vi "Get Username and Password.vi"(8 "error in":errorcluster, 11 "Item Ref in":T1 format="%.0x") -> (0 "error out":errorcluster, 1 "password":string, 2 "username":string, 3 "Item Ref out":T1 format="%.0x")   [LabVIEW 2024, in "SEECD System Explorer.lvlib"]
uses:
  NationalInstruments.VeriStand.SystemDefinitionAPI
  SEECD System Explorer.lvlib
  <vilib>/NI VeriStand/Custom Device Tools/Custom Device Utility Library/Custom Device Utility Library.lvlib
  <vilib>/NI VeriStand/Custom Device Offline API/Custom Device Offline API.lvlib
  <vilib>/NI VeriStand/Custom Device API/Custom Device Item Ref.ctl
  <vilib>/NI VeriStand/Custom Device API/Custom Device API.lvlib
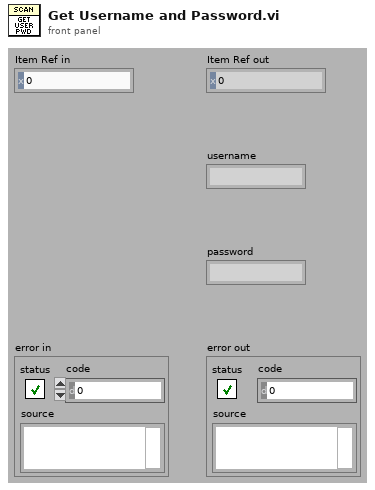
[diagram p1: front panel]
types:
  T1 = typedef "Custom Device API.lvlib/Custom Device Item Ref.ctl" = u64
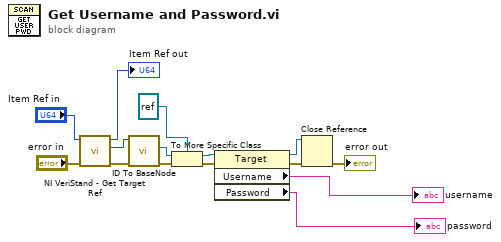
[diagram p0: block diagram]
diagram:
  n1 = call <vilib>:"NI VeriStand - Get Target Ref.vi"("error in"="error in", "Item Ref in"="Item Ref in") -> ("error out"=w2:errorcluster, "Target Ref"=w10:T1, "Item Ref out"=→"Item Ref out":T1)  [unwired: 6 in, 1 out]
  n2 = call <vilib>:"ID To BaseNode.vi"("error in (no error)"=w2, "ID in"=w10) -> ("error out"=w5:errorcluster, "BaseNode"=w4:refnum<k24>)  [unwired: 7 in, 1 out]
  n3 = To More Specific Class(target class=refnum<k24> refnum, reference=w4, error in=w5) -> (specific class reference=w6:refnum<k24>, error out=w7:errorcluster)
  n4 = property class="Target"(reference=w6, error in=w7) -> (reference out=w8:refnum<k24>, error out=w9:errorcluster, "Username"=→"username":string, "Password"=→"password":string)
  n5 = Close Reference(reference=w8, error in (no error)=w9) -> (error out=→"error out":errorcluster)
